vi "Get Market Summary.vi"(8 "error in":errorcluster) -> (0 "error out":errorcluster, 3 "Summary":T1)   [LabVIEW 2020, in "Full Featured MCP Server.lvlib"]
doc: "Returns a quick overview of the market: the average price change of all stocks over the last 60 seconds, the biggest gainer and the biggest loser of that minute, the mood of the market and how many news stories are unfolding right now."
uses:
  Full Featured MCP Server.lvlib
  Market/Market Mode.ctl
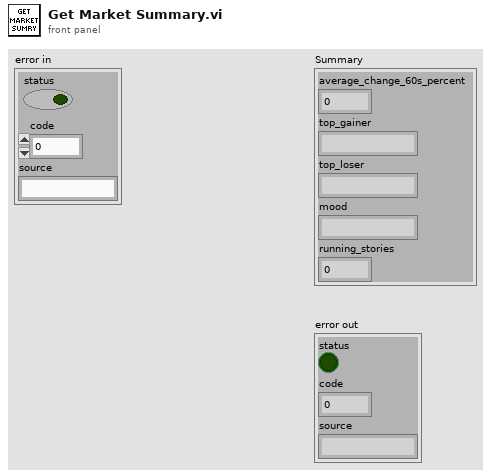
[diagram p1: front panel]
types:
  T1 = cluster{"average_change_60s_percent":dbl, "top_gainer":string, "top_loser":string, "mood":string, "running_stories":i32}
  T2 = typedef "Full Featured MCP Server.lvlib/Market Mode.ctl" = enum16{"Get", "Init", "Advance", "Buy", "Sell"}
  T3 = cluster{"tick":i32, "price history":dbl[][], "shock":dbl[], "momentum":dbl[], "nervousness":dbl[], "mood":dbl, "tension":dbl, "sector mood":dbl[], "news":cluster{"tick":i32, "headline":string, "stocks":i32[], "direction":string}[], "stories":cluster{"arc":i32, "step":i32, "due":i32, "stock":i32, "other":i32}[], "owned":i32[], "wallet":dbl}
  T4 = cluster{"arc":i32, "step":i32, "due":i32, "stock":i32, "other":i32}[]
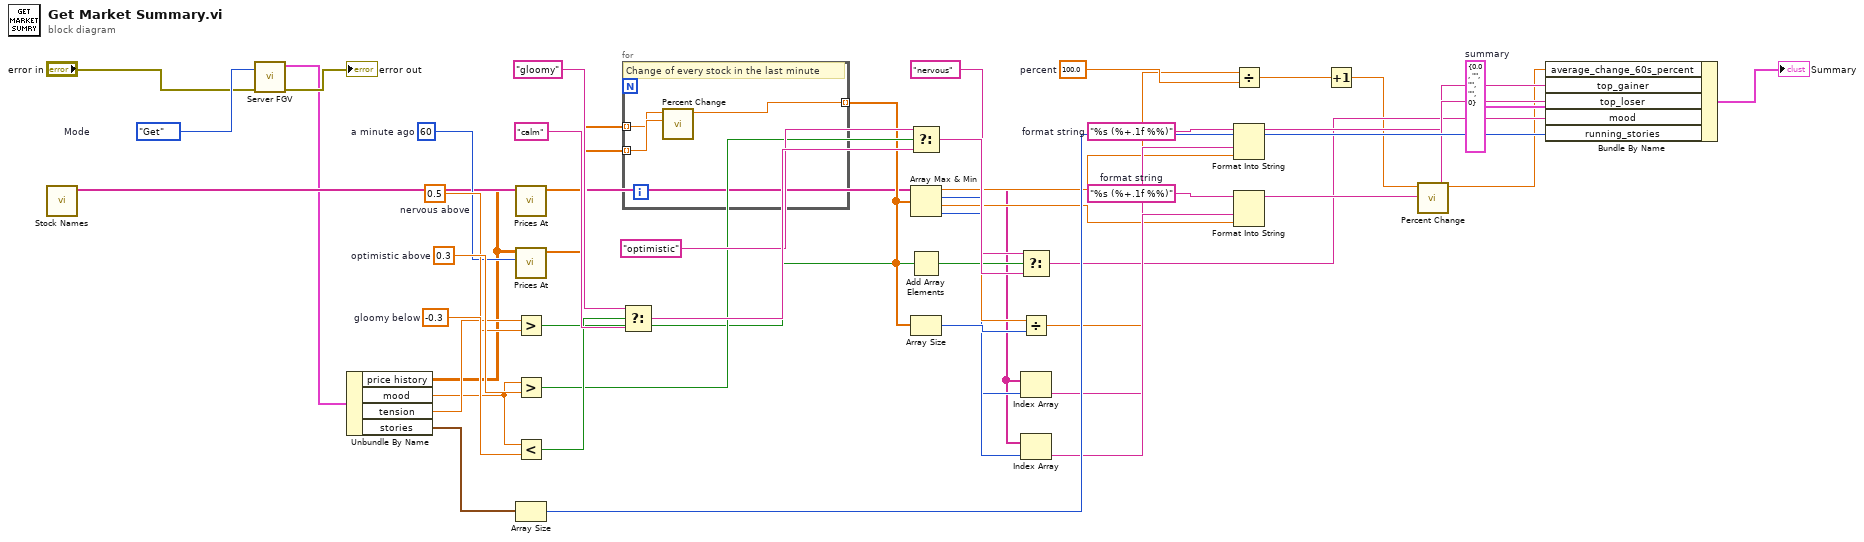
[diagram p0: block diagram]
diagram:
  w43 = "%s (%+.1f %%)"  # format string
  w40 = "%s (%+.1f %%)"  # format string
  w38 = T1 {"average_change_60s_percent"=0.0, "top_gainer"="", "top_loser"="", "mood"="", "running_stories"=0}  # summary
  w31 = -0.3  # gloomy below
  w28 = 0.3  # optimistic above
  w25 = 0.5  # nervous above
  w21 = 100.0  # percent
  w13 = 60  # a minute ago
  w2 = Market_Mode."Get"  # Mode
  n1 = call "Stock Names.vi"() -> ("names"=w9:string[])  [unwired: 11 in]
  n2 = call "Server FGV.vi"("Mode"=w2, "error in"="error in") -> ("error out"=→"error out":errorcluster, "market"=w3:T3)  [unwired: 7 in, 1 out]
  n3 = Unbundle By Name(w3) -> ("price history"=w5:dbl[][], "mood"=w6:dbl, "tension"=w7:dbl, "stories"=w8:T4)
  n4 = call "Prices At.vi"("price history"=w5) -> ("prices"=w10:dbl[])  [unwired: 10 in]
  n5 = call "Prices At.vi"("seconds ago"=w13, "price history"=w5) -> ("prices"=w11:dbl[])  [unwired: 9 in]
  n6 = Greater?(x=w7, y=w25) -> (0:w26:bool)
  n7 = Greater?(x=w6, y=w28) -> (0:w29:bool)
  n8 = Less?(x=w6, y=w31) -> (x < y?=w32:bool)
  n9 = Array Size(array=w8) -> (size(s)=w45:i32)
  n10 = for {
    tunnel: w10 -> [w47] mode=indexing
    tunnel: w11 -> [w48] mode=indexing
    tunnel: [w49] -> w12 mode=indexing
    # "Change of every stock in the last minute"
    n11 = call "Percent Change.vi"("before"=w48, "now"=w47) -> ("percent"=w49:dbl)  [unwired: 9 in]
  }
  n12 = Select(t="gloomy", s=w32, f="calm") -> (s? t:f=w35:string)
  n13 = Select(t="optimistic", s=w29, f=w35) -> (s? t:f=w36:string)
  n14 = Array Max & Min(array=w12) -> (max value=w14:dbl, max index (indices)=w15:i32, min value=w16:dbl, min index (indices)=w17:i32)
  n15 = Add Array Elements(numeric array=w12) -> (sum=w18:dbl)
  n16 = Array Size(array=w12) -> (size(s)=w19:i32)
  n17 = Select(t="nervous", s=w26, f=w36) -> (s? t:f=w37:string)
  n18 = Divide(x=w18, y=w19) -> (x/y=w20:dbl)
  n19 = Index Array(array=w9, index=w15) -> (element=w39:string)
  n20 = Index Array(array=w9, index=w17) -> (element=w42:string)
  n21 = Divide(x=w20, y=w21) -> (x/y=w22:dbl)
  n22 = Format Into String(format string=w40, w39, w14) -> (resulting string=w41:string)  [unwired: 2 in, 1 out]
  n23 = Format Into String(format string=w43, w42, w16) -> (resulting string=w44:string)  [unwired: 2 in, 1 out]
  n24 = Increment(x=w22) -> (x+1=w23:dbl)
  n25 = call "Percent Change.vi"("now"=w23) -> ("percent"=w24:dbl)  [unwired: 10 in]
  n26 = Bundle By Name(cluster=w38, "average_change_60s_percent"=w24, "top_gainer"=w41, "top_loser"=w44, "mood"=w37, "running_stories"=w45) -> (→"Summary":T1)
